vi "Read Sequence File.vi"(8 "error in":errorcluster, 11 "path":path) -> (0 "error out":errorcluster, 3 "Sequence File":T1)   [LabVIEW 2026]
doc: "Reads a sequence JSON file as text and parses it with Parse Sequence JSON.vi into a Sequence File cluster. An empty path returns error 7 instead of opening a file dialog; a missing file, a JSON error or an empty steps array (error 5001) is passed out on error out. AF-free."
uses:
  Typedefs/Step Config.ctl
  Typedefs/Sequence File.ctl
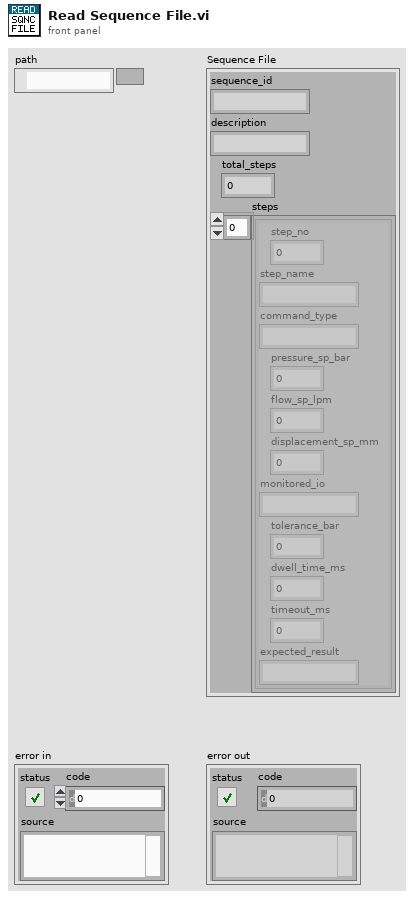
[diagram p1: front panel]
types:
  T1 = typedef "Sequence File.ctl" = cluster{"sequence_id":string, "description":string, "total_steps":i32, "steps":T2[]}
  T2 = typedef "Step Config.ctl" = cluster{"step_no":i32, "step_name":string, "command_type":string, "pressure_sp_bar":dbl, "flow_sp_lpm":dbl, "displacement_sp_mm":dbl, "monitored_io":string, "tolerance_bar":dbl, "dwell_time_ms":i32, "timeout_ms":i32, "expected_result":string}
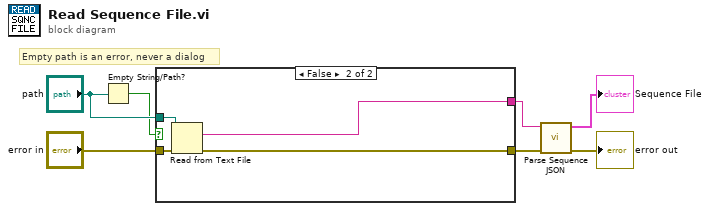
[diagram p0: block diagram]
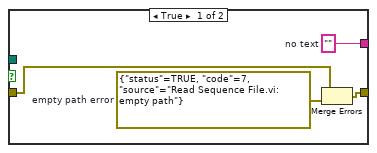
[diagram p2: hidden frame]
diagram:
  # "Empty path is an error, never a dialog"
  n1 = Empty String/Path?(string/path="path") -> (empty?=w5:bool)
  n2 = case shown="False" w5 {
    tunnel: "path" -> [_ w15]
    tunnel: "error in" -> [w11 w14]
    tunnel: [w9 w13] -> w4
    tunnel: [w8 w12] -> w3
    frame True {
      w9 = ""  # no text
      w10 = errorcluster {"status"=TRUE, "code"=7, "source"="Read Sequence File.vi: empty path"}  # empty path error
      n3 = Merge Errors(w11, w10) -> (w8:errorcluster)
    }
    frame False {
      n4 = Read from Text File(file (use dialog)=w15, error in=w14) -> (text=w13:string, error out=w12:errorcluster)  [unwired: 2 in, 2 out]
    }
  }
  n5 = call "Parse Sequence JSON.vi"("error in"=w3, "JSON string"=w4) -> ("error out"=→"error out":errorcluster, "Sequence File"=→"Sequence File":T1)  [unwired: 8 in]
